vi "Decode_Cmd.vi"(0 "Queue in":refnum<queue>, 1 "CycleStopReq in":bool, 3 "ExitReq in":bool, 4 "Paused in":bool, 6 "Array":bool[](array[boolean]), 7 "PrevDI":bool[](array[boolean])) -> (11 "ResetPB":bool, 12 "StartCmd":bool, 13 "Msg":string, 14 "CycleStopReq":bool, 15 "ExitReq out":bool, 17 "ResumeCmd":bool, 18 "PausedNow":bool, 19 "PausedNext":bool)   [LabVIEW 2018]
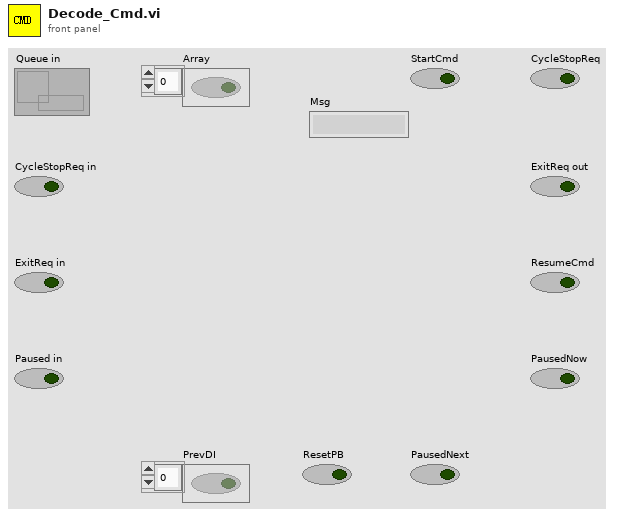
[diagram p1: front panel]
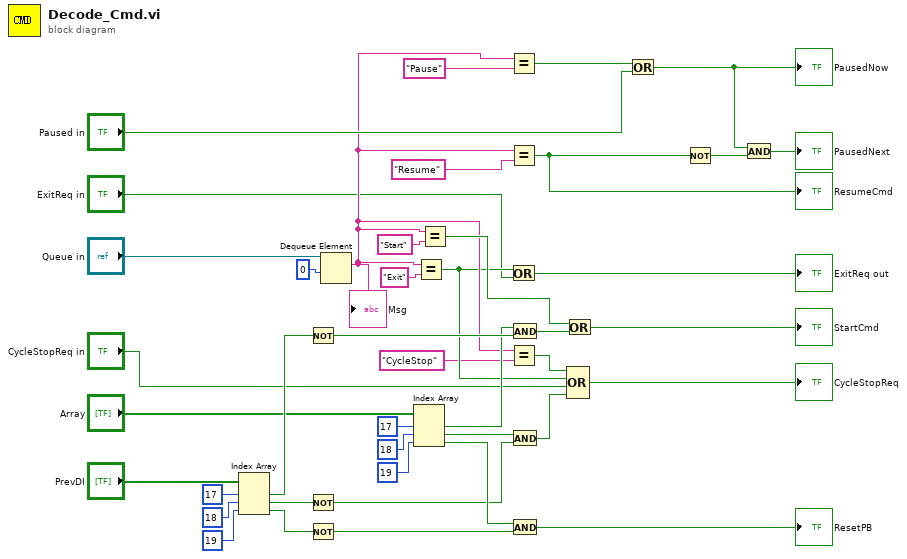
[diagram p0: block diagram]
diagram:
  n1 = Index Array(array="PrevDI", index #1=17 ("index"), index #2=18 ("index"), index #3=19 ("index")) -> (element #1=w28:bool, element #2=w31:bool, element #3=w34:bool)
  n2 = Not(x=w28) -> (.not. x?=w30:bool)
  n3 = Not(x=w31) -> (.not. x?=w33:bool)
  n4 = Not(x=w34) -> (.not. x?=w36:bool)
  n5 = Dequeue Element(queue="Queue in", timeout in ms (-1)=0) -> (element=w12:string)  [unwired: 1 in, 3 out]
  "Msg" <- w12
  n6 = Index Array(array="Array", index #1=17 ("index"), index #2=18 ("index"), index #3=19 ("index")) -> (element #1=w29:bool, element #2=w32:bool, element #3=w35:bool)
  n7 = Equal?(x=w12, y="Exit") -> (x = y?=w8:bool)
  n8 = Equal?(x=w12, y="Start") -> (x = y?=w37:bool)
  n9 = Equal?(x=w12, y="Pause") -> (x = y?=w18:bool)
  n10 = Equal?(x=w12, y="Resume") -> (x = y?=w19:bool)
  "ResumeCmd" <- w19
  n11 = Or(x=w8, y="ExitReq in") -> (x .or. y?=→"ExitReq out":bool)
  n12 = Equal?(x=w12, y="CycleStop") -> (x = y?=w7:bool)
  n13 = And(x=w29, y=w30) -> (x .and. y?=w38:bool)
  n14 = And(x=w32, y=w33) -> (x .and. y?=w40:bool)
  n15 = And(x=w35, y=w36) -> (x .and. y?=→"ResetPB":bool)
  n16 = Or(x=w37, y=w38) -> (x .or. y?=→"StartCmd":bool)
  n17 = Compound Arithmetic op=OR(w7, w8, "CycleStopReq in", w40) -> (→"CycleStopReq":bool)
  n18 = Or(x=w18, y="Paused in") -> (x .or. y?=w41:bool)
  "PausedNow" <- w41
  n19 = Not(x=w19) -> (.not. x?=w16:bool)
  n20 = And(x=w41, y=w16) -> (x .and. y?=→"PausedNext":bool)
